vi "MongoDB.FindOneByID.vi"(8 "error in (no error)":errorcluster, 10 "JSON Query String":string, 11 "MongoDB.Collection in":refnum<class "MongoDB.Collection.lvclass">) -> (0 "error out":errorcluster, 2 "Result":string, 3 "MongoDB.Collection out":refnum<class "MongoDB.Collection.lvclass">)   [LabVIEW 2014, in "MongoDB.Collection.lvclass"]
uses:
  MongoDB.Collection.lvclass
  C:/Users/Richard/Documents/GitHub/mongo-labview-driver/CSharp/bin/MongoDB.Bson.dll
  CSharp/bin/MongoDB.Bson.dll
  MongoDB.Collection.lvclass/MongoDB.Collection.ctl
  C:/Users/Richard/Documents/GitHub/mongo-labview-driver/CSharp/bin/MongoDB.Driver.Legacy.dll
  CSharp/bin/MongoDB.Driver.Legacy.dll
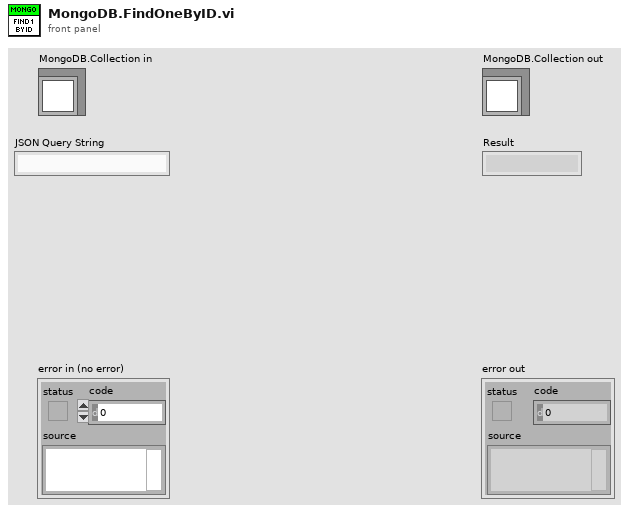
[diagram p1: front panel]
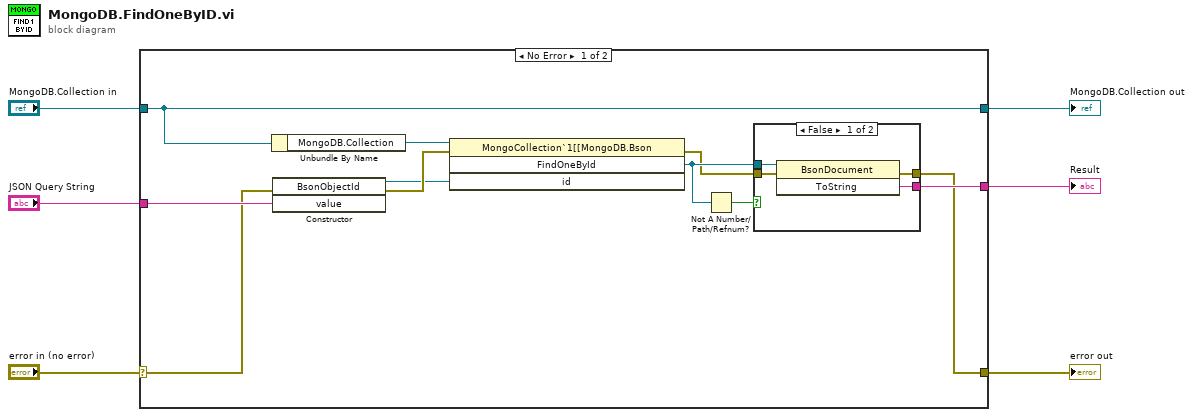
[diagram p0: block diagram]
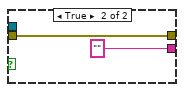
[diagram p2: hidden frame]
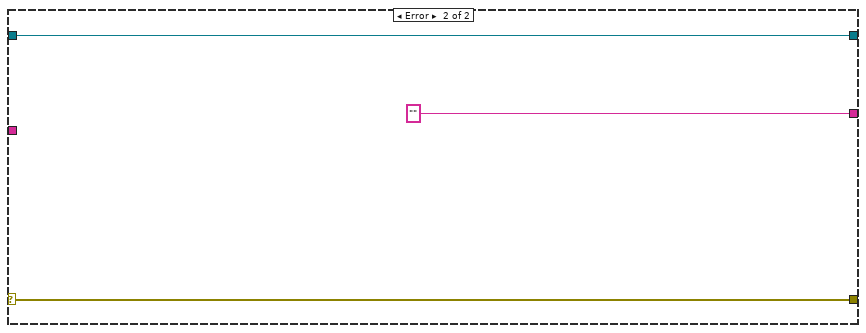
[diagram p3: hidden frame]
diagram:
  n1 = case shown="No Error" "error in (no error)" {
    selector: "error in (no error)" -> [w14 w26]
    tunnel: [w7 w26] -> w5
    tunnel: [w17 w25] -> w3
    tunnel: "MongoDB.Collection in" -> [w17 w25]
    tunnel: "JSON Query String" -> [w15 _]
    tunnel: [w8 "" ("ToString")] -> w1
    frame No Error {
      n2 = Unbundle By Name(w17) -> ("MongoDB.Collection"=w16:refnum<k24>)
      n3 = constructor class="BsonObjectId"(error in=w14, "value"=w15) -> (reference out=w11:refnum<k24>, error out=w13:errorcluster)  [unwired: 2 in, 2 out]
      n4 = invoke class="MongoCollection`1[[MongoDB.Bson" method="FindOneById"(reference=w16, error in=w13, "id"=w11) -> (error out=w9:errorcluster, "FindOneById"=w10:refnum<k24>)  [unwired: 1 in, 2 out]
      n5 = Not A Number/Path/Refnum?(number/path/refnum=w10) -> (NaN/Path/Refnum?=w12:bool)
      n6 = case shown="False" w12 {
        tunnel: [w21 "" ("AsString")] -> w8
        tunnel: w10 -> [w19 _]
        tunnel: w9 -> [w18 w22]
        tunnel: [w20 w22] -> w7
        frame False {
          n7 = invoke class="BsonDocument" method="ToString"(reference=w19, error in=w18) -> (error out=w20:errorcluster, "ToString"=w21:string)  [unwired: 1 in, 1 out]
        }
        frame True {
        }
      }
    }
    frame Error {
    }
  }
  "error out" <- w5
  "MongoDB.Collection out" <- w3
  "Result" <- w1
